vi "Pre-Build Custom Action.vi"(10 "Variant":variant) -> (0 "error out":errorcluster)   [LabVIEW 2021]
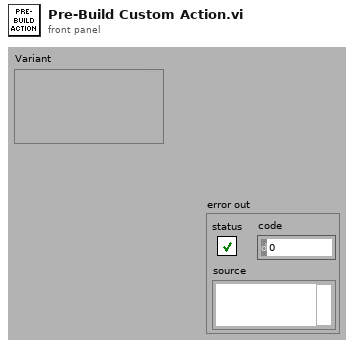
[diagram p1: front panel]
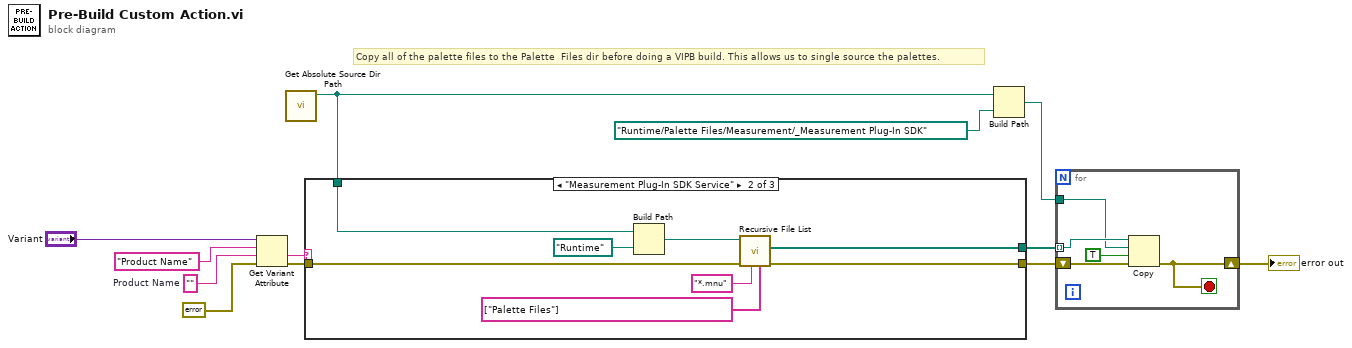
[diagram p0: block diagram]
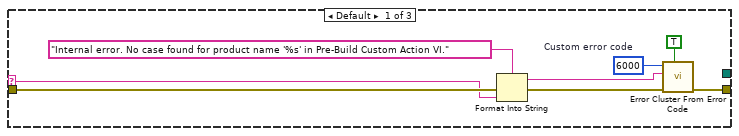
[diagram p2: hidden frame]
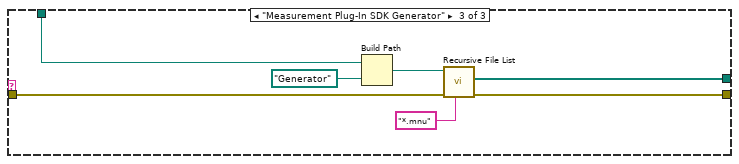
[diagram p3: hidden frame]
diagram:
  w11 = ""  # Product Name
  # "Copy all of the palette files to the Palette  Files dir before doing a VIPB build. This allows us to single source the palettes."
  n1 = Get Variant Attribute(Variant="Variant", name="Product Name", default value (empty Variant)=w11, error in=errorcluster {"status"=FALSE, "code"=0, "source"=""}) -> (value=w2:string, error out=w5:errorcluster)  [unwired: 2 out]
  n2 = call "Get Absolute Source Dir Path.vi"() -> ("source dir"=w1:path)  [unwired: 11 in]
  n3 = case shown="\"Measurement Plug-In SDK Service\"" w2 {
    selector: w2 -> [w13 _ _]
    tunnel: [_ w26 w34] -> w9
    tunnel: [w15 w25 w33] -> w8
    tunnel: w5 -> [w14 w24 w32]
    tunnel: w1 -> [_ w21 w29]
    frame Default {
      w19 = 6000  # Custom error code
      n4 = Format Into String(format string="Internal error. No case found for product name '%s' in Pre-Build Custom Action VI.", error in=w14, w13) -> (resulting string=w16:string, error out=w20:errorcluster)  [unwired: 1 in]
      n5 = call <vilib>:"Error Cluster From Error Code.vi"("show call chain? (False)"=TRUE, "error in (no error)"=w20, "error message (\"\")"=w16, "error code (0)"=w19) -> ("error out"=w15:errorcluster)  [unwired: 5 in]
    }
    frame "Measurement Plug-In SDK Service" {
      n6 = Build Path(base path=w21, name or relative path=path "Runtime") -> (appended path=w23:path)
      n7 = call <vilib>:"Recursive File List.vi"("Folders to Exclude"=string[] ["Palette Files"], "pattern"="*.mnu", "error in (no error)"=w24, "Folder Path"=w23) -> ("error out"=w25:errorcluster, "All Files in Dir"=w26:path[])  [unwired: 3 in, 3 out]
    }
    frame "Measurement Plug-In SDK Generator" {
      n8 = Build Path(base path=w29, name or relative path=path "Generator") -> (appended path=w30:path)
      n9 = call <vilib>:"Recursive File List.vi"("pattern"="*.mnu", "error in (no error)"=w32, "Folder Path"=w30) -> ("error out"=w33:errorcluster, "All Files in Dir"=w34:path[])  [unwired: 4 in, 3 out]
    }
  }
  n10 = Build Path(base path=w1, name or relative path=path "Runtime/Palette Files/Measurement/_Measurement Plug-In SDK") -> (appended path=w6:path)
  n11 = for {
    tunnel: w9 -> [w38] mode=indexing
    tunnel: w6 -> [w37]
    shift-right: [w36] -> w4
    shift-left: w8 -> [w40]
    stop <- w36 stop-if-true
    n12 = Copy(8:w40, 9:TRUE ("overwrite (F)"), 10:w37, 11:w38) -> (0:w36:errorcluster)  [unwired: 1 in, 2 out]
  }
  "error out" <- w4
